vi "Write CE BTLE Power Setting.vi"(8 "error in (no error)":errorcluster, 10 "CE BTLE Power Setting":T1 {"Center and Span Frequency(Hz)"."Span" format="%#_6p"; "Center and Span Frequency(Hz)"."Center" format="%#_6p"}, 11 "SA Measurement in":refnum<class "SA Measurement.lvclass">) -> (0 "error out":errorcluster, 3 "SA Measurement out":refnum<class "SA Measurement.lvclass">)   [LabVIEW 2023, in "Spectrum Analyzer.lvlib" / "SA Measurement.lvclass"]
uses:
  SA Measurement.lvclass
  TYPE DEFINITION/SA Measurement Class/TYPE CE BTLE Power Setting Parameter.ctl
  TYPE DEFINITION/TYPE Center and Span Frequency.ctl
  TYPE DEFINITION/TYPE Reference Level and Atten Param.ctl
  SA Measurement.lvclass/SA Measurement.ctl
  Spectrum Analyzer.lvlib
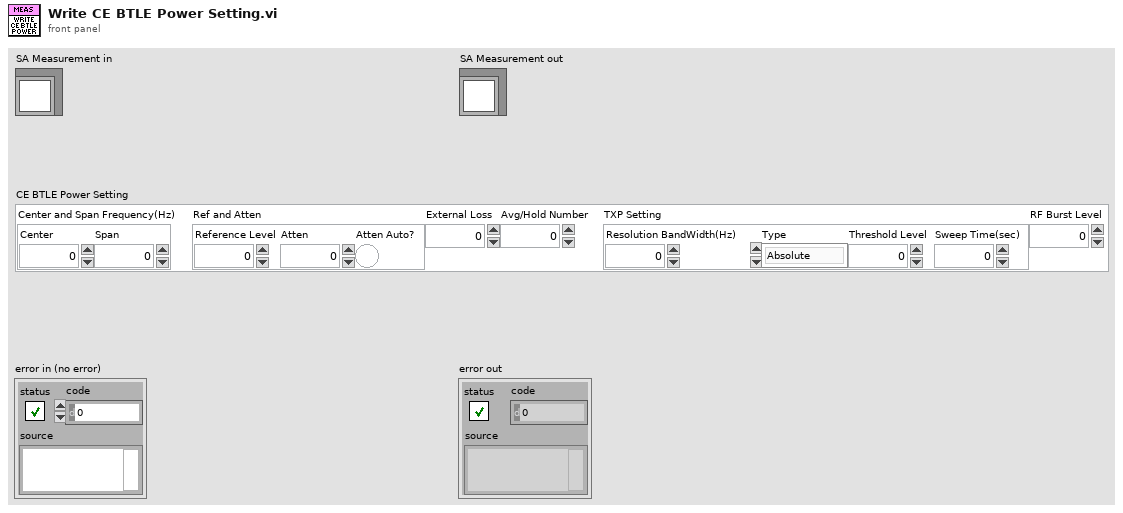
[diagram p1: front panel]
types:
  T1 = typedef "Spectrum Analyzer.lvlib/TYPE CE BTLE Power Setting Parameter.ctl" = cluster{"Center and Span Frequency(Hz)":T2, "Ref and Atten":T3, "External Loss":dbl, "Avg/Hold Number":u32, "TXP Setting":cluster{"Resolution BandWidth(Hz)":dbl, "Type":enum16{"Absolute", "Relative"}, "Threshold Level":dbl, "Sweep Time(sec)":dbl}, "RF Burst Level":dbl}
  T2 = typedef "Spectrum Analyzer.lvlib/TYPE Center and Span Frequency.ctl" = cluster{"Center":dbl, "Span":dbl}
  T3 = typedef "Spectrum Analyzer.lvlib/TYPE Reference Level and Atten Param.ctl" = cluster{"Reference Level":dbl, "Atten":i32, "Atten Auto?":bool}
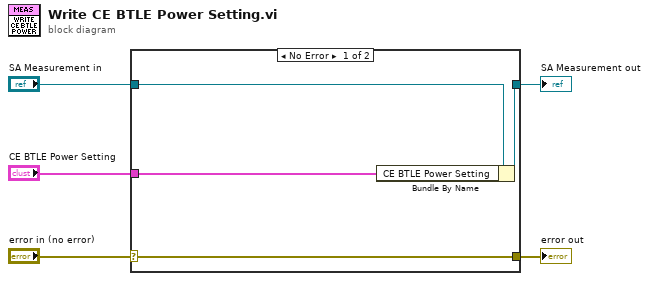
[diagram p0: block diagram]
diagram:
  n1 = case shown="No Error" "error in (no error)" {
    selector: "error in (no error)" -> [w9 w10]
    tunnel: [w9 w10] -> w4
    tunnel: [w7 w11] -> w2
    tunnel: "SA Measurement in" -> [w8 w11]
    tunnel: "CE BTLE Power Setting" -> [w6 _]
    frame No Error {
      n2 = Bundle By Name(cluster=w8, "CE BTLE Power Setting"=w6) -> (w7:refnum<class "SA Measurement.lvclass">)
    }
    frame Error {
    }
  }
  "error out" <- w4
  "SA Measurement out" <- w2
